vi "Interlock messages.vi"(0 "Fault bits":u32) -> (15 "Messages":string)   [LabVIEW 2025]
doc: "Decode every set permissive or fault bit in priority order."
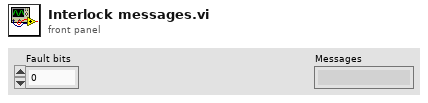
[diagram p1: front panel]
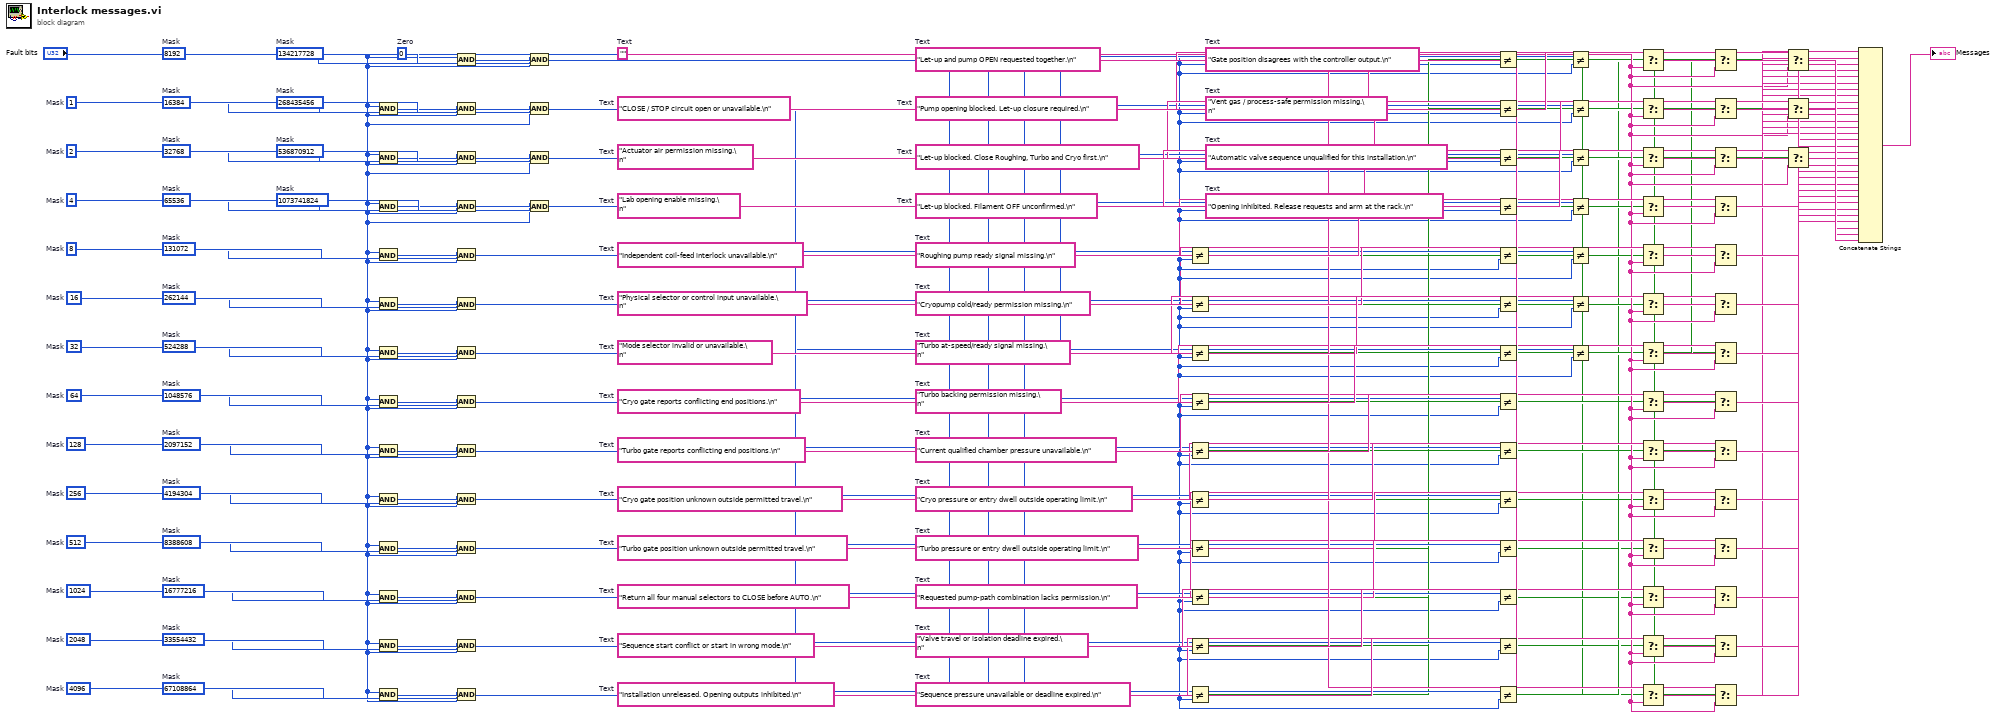
[diagram p0: block diagram]
diagram:
  w157 = "Opening inhibited. Release requests and arm at the rack.\n"  # Text
  w155 = "Automatic valve sequence unqualified for this installation.\n"  # Text
  w153 = "Vent gas / process-safe permission missing.\n"  # Text
  w151 = "Gate position disagrees with the controller output.\n"  # Text
  w149 = "Sequence pressure unavailable or deadline expired.\n"  # Text
  w147 = "Valve travel or isolation deadline expired.\n"  # Text
  w145 = "Requested pump-path combination lacks permission.\n"  # Text
  w143 = "Turbo pressure or entry dwell outside operating limit.\n"  # Text
  w141 = "Cryo pressure or entry dwell outside operating limit.\n"  # Text
  w139 = "Current qualified chamber pressure unavailable.\n"  # Text
  w137 = "Turbo backing permission missing.\n"  # Text
  w135 = "Turbo at-speed/ready signal missing.\n"  # Text
  w133 = "Cryopump cold/ready permission missing.\n"  # Text
  w131 = "Roughing pump ready signal missing.\n"  # Text
  w129 = "Let-up blocked. Filament OFF unconfirmed.\n"  # Text
  w127 = "Let-up blocked. Close Roughing, Turbo and Cryo first.\n"  # Text
  w125 = "Pump opening blocked. Let-up closure required.\n"  # Text
  w123 = "Let-up and pump OPEN requested together.\n"  # Text
  w121 = "Installation unreleased. Opening outputs inhibited.\n"  # Text
  w119 = "Sequence start conflict or start in wrong mode.\n"  # Text
  w117 = "Return all four manual selectors to CLOSE before AUTO.\n"  # Text
  w115 = "Turbo gate position unknown outside permitted travel.\n"  # Text
  w113 = "Cryo gate position unknown outside permitted travel.\n"  # Text
  w111 = "Turbo gate reports conflicting end positions.\n"  # Text
  w109 = "Cryo gate reports conflicting end positions.\n"  # Text
  w107 = "Mode selector invalid or unavailable.\n"  # Text
  w105 = "Physical selector or control input unavailable.\n"  # Text
  w103 = "Independent coil-feed interlock unavailable.\n"  # Text
  w101 = "Lab opening enable missing.\n"  # Text
  w99 = "Actuator air permission missing.\n"  # Text
  w97 = "CLOSE / STOP circuit open or unavailable.\n"  # Text
  w96 = ""  # Text
  w93 = u32 1073741824  # Mask
  w90 = u32 536870912  # Mask
  w87 = u32 268435456  # Mask
  w84 = u32 134217728  # Mask
  w81 = u32 67108864  # Mask
  w78 = u32 33554432  # Mask
  w75 = u32 16777216  # Mask
  w72 = u32 8388608  # Mask
  w69 = u32 4194304  # Mask
  w66 = u32 2097152  # Mask
  w63 = u32 1048576  # Mask
  w60 = u32 524288  # Mask
  w57 = u32 262144  # Mask
  w54 = u32 131072  # Mask
  w51 = u32 65536  # Mask
  w48 = u32 32768  # Mask
  w45 = u32 16384  # Mask
  w42 = u32 8192  # Mask
  w39 = u32 4096  # Mask
  w36 = u32 2048  # Mask
  w33 = u32 1024  # Mask
  w30 = u32 512  # Mask
  w27 = u32 256  # Mask
  w24 = u32 128  # Mask
  w21 = u32 64  # Mask
  w18 = u32 32  # Mask
  w15 = u32 16  # Mask
  w12 = u32 8  # Mask
  w9 = u32 4  # Mask
  w6 = u32 2  # Mask
  w3 = u32 1  # Mask
  w2 = u32 0  # Zero
  n1 = And(x="Fault bits", y=w3) -> (x .and. y?=w4:u32)
  n2 = And(x="Fault bits", y=w6) -> (x .and. y?=w7:u32)
  n3 = And(x="Fault bits", y=w9) -> (x .and. y?=w10:u32)
  n4 = And(x="Fault bits", y=w12) -> (x .and. y?=w13:u32)
  n5 = And(x="Fault bits", y=w15) -> (x .and. y?=w16:u32)
  n6 = And(x="Fault bits", y=w18) -> (x .and. y?=w19:u32)
  n7 = And(x="Fault bits", y=w21) -> (x .and. y?=w22:u32)
  n8 = And(x="Fault bits", y=w24) -> (x .and. y?=w25:u32)
  n9 = And(x="Fault bits", y=w27) -> (x .and. y?=w28:u32)
  n10 = And(x="Fault bits", y=w30) -> (x .and. y?=w31:u32)
  n11 = And(x="Fault bits", y=w33) -> (x .and. y?=w34:u32)
  n12 = And(x="Fault bits", y=w36) -> (x .and. y?=w37:u32)
  n13 = And(x="Fault bits", y=w39) -> (x .and. y?=w40:u32)
  n14 = And(x="Fault bits", y=w42) -> (x .and. y?=w43:u32)
  n15 = And(x="Fault bits", y=w45) -> (x .and. y?=w46:u32)
  n16 = And(x="Fault bits", y=w48) -> (x .and. y?=w49:u32)
  n17 = And(x="Fault bits", y=w51) -> (x .and. y?=w52:u32)
  n18 = And(x="Fault bits", y=w54) -> (x .and. y?=w55:u32)
  n19 = And(x="Fault bits", y=w57) -> (x .and. y?=w58:u32)
  n20 = And(x="Fault bits", y=w60) -> (x .and. y?=w61:u32)
  n21 = And(x="Fault bits", y=w63) -> (x .and. y?=w64:u32)
  n22 = And(x="Fault bits", y=w66) -> (x .and. y?=w67:u32)
  n23 = And(x="Fault bits", y=w69) -> (x .and. y?=w70:u32)
  n24 = And(x="Fault bits", y=w72) -> (x .and. y?=w73:u32)
  n25 = And(x="Fault bits", y=w75) -> (x .and. y?=w76:u32)
  n26 = And(x="Fault bits", y=w78) -> (x .and. y?=w79:u32)
  n27 = And(x="Fault bits", y=w81) -> (x .and. y?=w82:u32)
  n28 = And(x="Fault bits", y=w84) -> (x .and. y?=w85:u32)
  n29 = And(x="Fault bits", y=w87) -> (x .and. y?=w88:u32)
  n30 = And(x="Fault bits", y=w90) -> (x .and. y?=w91:u32)
  n31 = And(x="Fault bits", y=w93) -> (x .and. y?=w94:u32)
  n32 = Not Equal?(x=w4, y=w2) -> (x != y?=w5:bool)
  n33 = Not Equal?(x=w7, y=w2) -> (x != y?=w8:bool)
  n34 = Not Equal?(x=w10, y=w2) -> (x != y?=w11:bool)
  n35 = Not Equal?(x=w13, y=w2) -> (x != y?=w14:bool)
  n36 = Not Equal?(x=w16, y=w2) -> (x != y?=w17:bool)
  n37 = Not Equal?(x=w19, y=w2) -> (x != y?=w20:bool)
  n38 = Not Equal?(x=w22, y=w2) -> (x != y?=w23:bool)
  n39 = Not Equal?(x=w25, y=w2) -> (x != y?=w26:bool)
  n40 = Not Equal?(x=w28, y=w2) -> (x != y?=w29:bool)
  n41 = Not Equal?(x=w31, y=w2) -> (x != y?=w32:bool)
  n42 = Not Equal?(x=w34, y=w2) -> (x != y?=w35:bool)
  n43 = Not Equal?(x=w37, y=w2) -> (x != y?=w38:bool)
  n44 = Not Equal?(x=w40, y=w2) -> (x != y?=w41:bool)
  n45 = Not Equal?(x=w43, y=w2) -> (x != y?=w44:bool)
  n46 = Not Equal?(x=w46, y=w2) -> (x != y?=w47:bool)
  n47 = Not Equal?(x=w49, y=w2) -> (x != y?=w50:bool)
  n48 = Not Equal?(x=w52, y=w2) -> (x != y?=w53:bool)
  n49 = Not Equal?(x=w55, y=w2) -> (x != y?=w56:bool)
  n50 = Not Equal?(x=w58, y=w2) -> (x != y?=w59:bool)
  n51 = Not Equal?(x=w61, y=w2) -> (x != y?=w62:bool)
  n52 = Not Equal?(x=w64, y=w2) -> (x != y?=w65:bool)
  n53 = Not Equal?(x=w67, y=w2) -> (x != y?=w68:bool)
  n54 = Not Equal?(x=w70, y=w2) -> (x != y?=w71:bool)
  n55 = Not Equal?(x=w73, y=w2) -> (x != y?=w74:bool)
  n56 = Not Equal?(x=w76, y=w2) -> (x != y?=w77:bool)
  n57 = Not Equal?(x=w79, y=w2) -> (x != y?=w80:bool)
  n58 = Not Equal?(x=w82, y=w2) -> (x != y?=w83:bool)
  n59 = Not Equal?(x=w85, y=w2) -> (x != y?=w86:bool)
  n60 = Not Equal?(x=w88, y=w2) -> (x != y?=w89:bool)
  n61 = Not Equal?(x=w91, y=w2) -> (x != y?=w92:bool)
  n62 = Not Equal?(x=w94, y=w2) -> (x != y?=w95:bool)
  n63 = Select(t=w97, s=w5, f=w96) -> (s? t:f=w98:string)
  n64 = Select(t=w99, s=w8, f=w96) -> (s? t:f=w100:string)
  n65 = Select(t=w101, s=w11, f=w96) -> (s? t:f=w102:string)
  n66 = Select(t=w103, s=w14, f=w96) -> (s? t:f=w104:string)
  n67 = Select(t=w105, s=w17, f=w96) -> (s? t:f=w106:string)
  n68 = Select(t=w107, s=w20, f=w96) -> (s? t:f=w108:string)
  n69 = Select(t=w109, s=w23, f=w96) -> (s? t:f=w110:string)
  n70 = Select(t=w111, s=w26, f=w96) -> (s? t:f=w112:string)
  n71 = Select(t=w113, s=w29, f=w96) -> (s? t:f=w114:string)
  n72 = Select(t=w115, s=w32, f=w96) -> (s? t:f=w116:string)
  n73 = Select(t=w117, s=w35, f=w96) -> (s? t:f=w118:string)
  n74 = Select(t=w119, s=w38, f=w96) -> (s? t:f=w120:string)
  n75 = Select(t=w121, s=w41, f=w96) -> (s? t:f=w122:string)
  n76 = Select(t=w123, s=w44, f=w96) -> (s? t:f=w124:string)
  n77 = Select(t=w125, s=w47, f=w96) -> (s? t:f=w126:string)
  n78 = Select(t=w127, s=w50, f=w96) -> (s? t:f=w128:string)
  n79 = Select(t=w129, s=w53, f=w96) -> (s? t:f=w130:string)
  n80 = Select(t=w131, s=w56, f=w96) -> (s? t:f=w132:string)
  n81 = Select(t=w133, s=w59, f=w96) -> (s? t:f=w134:string)
  n82 = Select(t=w135, s=w62, f=w96) -> (s? t:f=w136:string)
  n83 = Select(t=w137, s=w65, f=w96) -> (s? t:f=w138:string)
  n84 = Select(t=w139, s=w68, f=w96) -> (s? t:f=w140:string)
  n85 = Select(t=w141, s=w71, f=w96) -> (s? t:f=w142:string)
  n86 = Select(t=w143, s=w74, f=w96) -> (s? t:f=w144:string)
  n87 = Select(t=w145, s=w77, f=w96) -> (s? t:f=w146:string)
  n88 = Select(t=w147, s=w80, f=w96) -> (s? t:f=w148:string)
  n89 = Select(t=w149, s=w83, f=w96) -> (s? t:f=w150:string)
  n90 = Select(t=w151, s=w86, f=w96) -> (s? t:f=w152:string)
  n91 = Select(t=w153, s=w89, f=w96) -> (s? t:f=w154:string)
  n92 = Select(t=w155, s=w92, f=w96) -> (s? t:f=w156:string)
  n93 = Select(t=w157, s=w95, f=w96) -> (s? t:f=w158:string)
  n94 = Concatenate Strings(w98, w100, w102, w104, w106, w108, w110, w112, w114, w116, w118, w120, w122, w124, w126, w128, w130, w132, w134, w136, w138, w140, w142, w144, w146, w148, w150, w152, w154, w156, w158) -> (→"Messages":string)
